vi "Write Microscope Metadata.vi"(0 "File Path":path, 11 "Error In":errorcluster) -> (4 "File Path (Dup)":path, 15 "Write Errror":errorcluster)   [LabVIEW 2016]
uses:
  Microscope Modules/4Pi Capture Manager/4Pi Capture Manager Controls/4Pi Capture Notifier Type.ctl
  Microscope Modules/4Pi Capture Manager/4Pi Capture Manager Controls/4Pi Capture Actions.ctl
  Microscope Modules/4Pi Capture Manager/4Pi Capture Manager Controls/4Pi Capture Switch Line Scan Modes.ctl
  Microscope Modules/Orca Flash Capture Manager/Orca Flash Capture Manager Controls/Orca Flash Capture Notifier Type.ctl
  Microscope Modules/Orca Flash Capture Manager/Orca Flash Capture Manager Controls/Orca Flash Capture Actions.ctl
  Microscope Modules/Orca Flash Capture Manager/Orca Flash Capture Manager Controls/Orca Flash Capture Switch Line Scan Modes.ctl
  Device Metadata Types/Capture Metadata.ctl
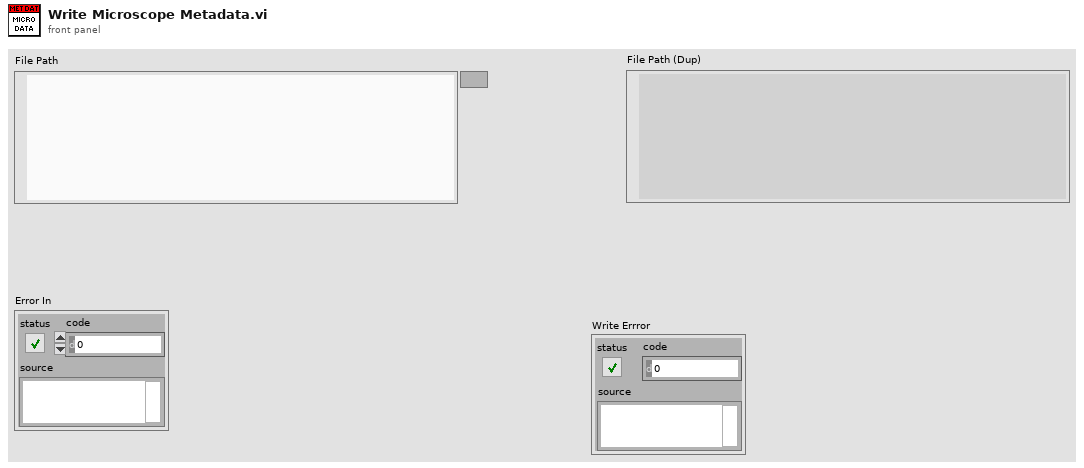
[diagram p1: front panel]
types:
  T1 = typedef "Capture Metadata.ctl" = cluster{"Capture_Exposure_sec":dbl, "Cycles":u16, "Frames":u32, "No_of_Z_Steps":u16, "Z_Step_Size_um":dbl, "Init_Z_Position_um":dbl, "Save_Path":string, "Line_Scan":bool, "Line_Scan_Mode":string, "channelCode":u8, "setupName":string}
  T2 = typedef "Orca Flash Capture Notifier Type.ctl" = cluster{"Actions":T3, "Running?":bool, "Preview Exposure (s)":dbl, "Capture Exposure (s)":dbl, "Cycles":u16, "Frames":u32, "No. of Z Steps":u16, "Z Step Size (µm)":dbl, "Base Path":path, "Init Z Position (µm)":dbl, "Lasers Lines":string[], "Save Path":path, "Line Scan?":bool, "Line Scan Mode":T4, "Collect Metadata?":bool, "channelCode":u8, "setupName":string}
  T3 = typedef "Orca Flash Capture Actions.ctl" = enum16{"Idle", "Live Preview", "Capture", "Check File Name", "Laser On", "Laser Off", "Open Shutters", "Close Shutters", "Set Exposure Time", "Start Acquisition", "Update SubFolder", "Write Metadata", "Setup", "Camera", "Switch", "Step", "Cycle", "External Cycle Sync", "Abort", "Quit"}
  T4 = typedef "Orca Flash Capture Switch Line Scan Modes.ctl" = enum32{"Automatic", "Use Presets", "Manual"}
  T5 = typedef "4Pi Capture Notifier Type.ctl" = cluster{"Actions":T6, "Running?":bool, "Preview Exposure (s)":dbl, "Capture Exposure (s)":dbl, "Cycles":u16, "Frames":u32, "No. of Z Steps":u16, "Z Step Size (µm)":dbl, "Base Path":path, "Init Z Position (µm)":dbl, "Lasers Lines":string[], "Save Path":path, "Line Scan?":bool, "Line Scan Mode":T7, "Metadata File Ref":refnum<file>}
  T6 = typedef "4Pi Capture Actions.ctl" = enum16{"Idle", "Live Preview", "Capture", "Laser On", "Laser Off", "Open Shutters", "Close Shutters", "Set Exposure Time", "Start Acquisition", "Update SubFolder", "Setup", "Camera", "Switch", "Step", "Cycle", "External Cycle Sync", "Write Metadata", "Abort", "Quit"}
  T7 = typedef "4Pi Capture Switch Line Scan Modes.ctl" = enum32{"Automatic", "Use Presets", "Manual"}
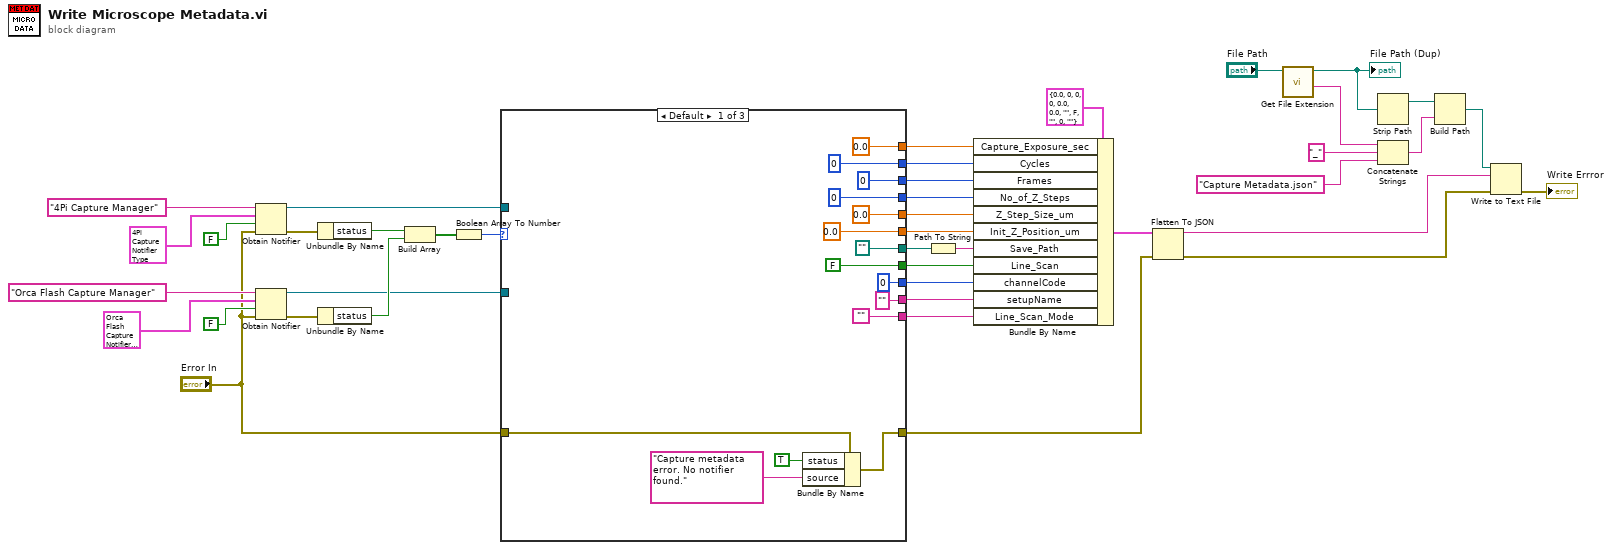
[diagram p0: block diagram]
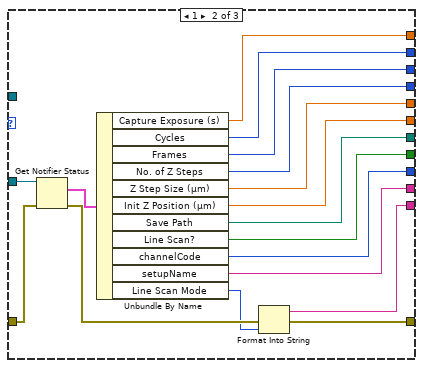
[diagram p2: hidden frame]
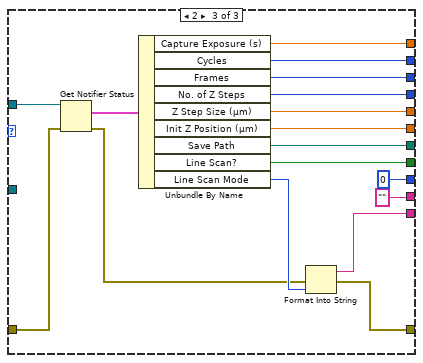
[diagram p3: hidden frame]
diagram:
  n1 = Obtain Notifier(name (unnamed)="4Pi Capture Manager", notification data type=T5 {"Actions"=enum."Live Preview", "Running?"=FALSE, "Preview Exposure (s)"=0.1, "Capture Exposure (s)"=0.1, "Cycles"=1, "Frames"=0, "No. of Z Steps"=0, "Z Step Size (µm)"=0.0, "Base Path"=path "", "Init Z Position (µm)"=0.0, "Lasers Lines"=[], "Save Path"=path "", "Line Scan?"=FALSE, "Line Scan Mode"=enum."Automatic", "Metadata File Ref"=refnum} ("4Pi Capture Notifier Type"), create if not found? (T)=FALSE, error in (no error)="Error In") -> (notifier out=w23:refnum<notifier>, error out=w29:errorcluster)  [unwired: 1 out]
  n2 = Obtain Notifier(name (unnamed)="Orca Flash Capture Manager", notification data type=T2 {"Actions"=enum."Live Preview", "Running?"=FALSE, "Preview Exposure (s)"=0.1, "Capture Exposure (s)"=0.1, "Cycles"=1, "Frames"=0, "No. of Z Steps"=0, "Z Step Size (µm)"=0.0, "Base Path"=path "", "Init Z Position (µm)"=0.0, "Lasers Lines"=[], "Save Path"=path "", "Line Scan?"=FALSE, "Line Scan Mode"=enum."Automatic", "Collect Metadata?"=FALSE, "channelCode"=0, "setupName"=""} ("4Pi Capture Notifier Type"), create if not found? (T)=FALSE, error in (no error)="Error In") -> (notifier out=w22:refnum<notifier>, error out=w28:errorcluster)  [unwired: 1 out]
  n3 = Unbundle By Name(w29) -> ("status"=w27:bool)
  n4 = Unbundle By Name(w28) -> ("status"=w26:bool)
  n5 = Build Array(w27, w26) -> (w25:bool[])
  n6 = Boolean Array To Number(Boolean array=w25) -> (number=w24:u32)
  n7 = case shown="Default" w24 {
    tunnel: w23 -> [_ _ w90]
    tunnel: w22 -> [_ w73 _]
    tunnel: [0.0 ("Capture Exposure (s)") w71 w88] -> w19
    tunnel: [u16 0 ("Cycles") w70 w87] -> w18
    tunnel: [u32 0 ("Frames") w69 w86] -> w17
    tunnel: [u16 0 ("No. of Z Steps") w68 w85] -> w16
    tunnel: [0.0 ("Z Step Size (µm)") w67 w84] -> w15
    tunnel: [0.0 ("Init Z Position (µm)") w66 w83] -> w14
    tunnel: [path "" w65 w82] -> w13
    tunnel: [FALSE ("Line Scan?") w64 w81] -> w11
    tunnel: ["" w63 w79] -> w3
    tunnel: "Error In" -> [w47 w61 w77]
    tunnel: [w44 w62 w78] -> w9
    tunnel: [u8 0 ("channelCode") w58 u8 0 ("channelCode")] -> w2
    tunnel: ["" ("setupName") w57 "" ("setupName")] -> w1
    frame Default {
      n8 = Bundle By Name(cluster=w47, "status"=TRUE, "source"="Capture metadata error. No notifier found.") -> (w44:errorcluster)
    }
    frame 1 {
      n9 = Get Notifier Status(notifier=w73, error in (no error)=w61) -> (current notification=w72:T2, error out=w60:errorcluster)  [unwired: 3 out]
      n10 = Unbundle By Name(w72) -> ("Capture Exposure (s)"=w71:dbl, "Cycles"=w70:u16, "Frames"=w69:u32, "No. of Z Steps"=w68:u16, "Z Step Size (µm)"=w67:dbl, "Init Z Position (µm)"=w66:dbl, "Save Path"=w65:path, "Line Scan?"=w64:bool, "channelCode"=w58:u8, "setupName"=w57:string, "Line Scan Mode"=w59:T4)
      n11 = Format Into String(error in=w60, w59) -> (resulting string=w63:string, error out=w62:errorcluster)  [unwired: 2 in]
    }
    frame 2 {
      n12 = Get Notifier Status(notifier=w90, error in (no error)=w77) -> (current notification=w89:T5, error out=w76:errorcluster)  [unwired: 3 out]
      n13 = Unbundle By Name(w89) -> ("Capture Exposure (s)"=w88:dbl, "Cycles"=w87:u16, "Frames"=w86:u32, "No. of Z Steps"=w85:u16, "Z Step Size (µm)"=w84:dbl, "Init Z Position (µm)"=w83:dbl, "Save Path"=w82:path, "Line Scan?"=w81:bool, "Line Scan Mode"=w80:T7)
      n14 = Format Into String(error in=w76, w80) -> (resulting string=w79:string, error out=w78:errorcluster)  [unwired: 2 in]
    }
  }
  n15 = Path To String(path=w13) -> (string=w12:string)
  n16 = Bundle By Name(cluster=T1 {"Capture_Exposure_sec"=0.0, "Cycles"=0, "Frames"=0, "No_of_Z_Steps"=0, "Z_Step_Size_um"=0.0, "Init_Z_Position_um"=0.0, "Save_Path"="", "Line_Scan"=FALSE, "Line_Scan_Mode"="", "channelCode"=0, "setupName"=""} ("4Pi Capture Notifier Type"), "Capture_Exposure_sec"=w19, "Cycles"=w18, "Frames"=w17, "No_of_Z_Steps"=w16, "Z_Step_Size_um"=w15, "Init_Z_Position_um"=w14, "Save_Path"=w12, "Line_Scan"=w11, "channelCode"=w2, "setupName"=w1, "Line_Scan_Mode"=w3) -> (w20:T1)
  n17 = Flatten To JSON(anything=w20, error in (no error)=w9) -> (JSON string=w8:string, 11:w7:errorcluster)  [unwired: 1 in]
  n18 = call <vilib>:"Get File Extension.vi"("file"="File Path") -> ("filename without extension"=w4:string, "dup file"=w5:path)  [unwired: 6 in, 3 out]
  "File Path (Dup)" <- w5
  n19 = Strip Path(path=w5) -> (stripped path=w41:path)  [unwired: 1 out]
  n20 = Concatenate Strings(w4, "_" ("string"), "Capture Metadata.json" ("name or relative path")) -> (w38:string)
  n21 = Build Path(base path=w41, name or relative path=w38) -> (appended path=w37:path)
  n22 = Write to Text File(file (use dialog)=w37, text=w8, error in=w7) -> (error out=→"Write Errror":errorcluster)  [unwired: 1 in, 2 out]
